vi "measure BT Frequency Separation Step2.vi"(8 "error in (no error)":errorcluster, 11 "SA Measurement in":refnum<class "SA Measurement.lvclass">) -> (0 "error out":errorcluster, 3 "SA Measurement out":refnum<class "SA Measurement.lvclass">)   [LabVIEW 2023, in "Spectrum Analyzer.lvlib" / "SA Measurement.lvclass"]
uses:
  SA Measurement.lvclass
  SA Measurement.lvclass/SA Measurement.ctl
  TYPE DEFINITION/TYPE Marker Peak Search Type.ctl
  Spectrum Analyzer.lvlib
  Interface_Spectrum/Interface_Spectrum.lvclass
  TYPE DEFINITION/TYPE Marker Control Mode.ctl
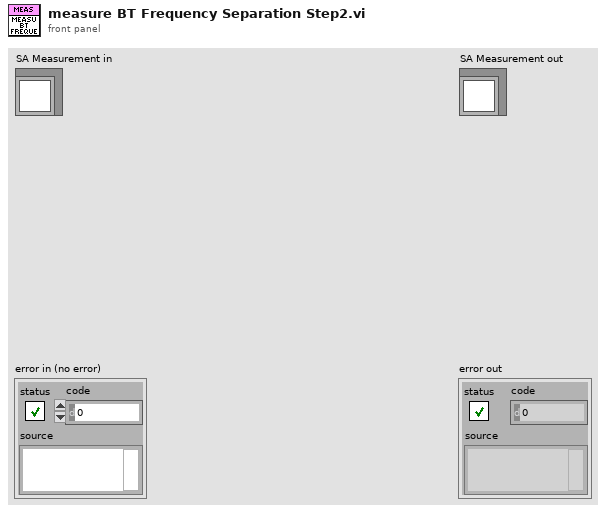
[diagram p1: front panel]
types:
  T1 = typedef "Spectrum Analyzer.lvlib/TYPE Marker Peak Search Type.ctl" = enum16{"Max", "Next Peak"}
  T2 = typedef "Spectrum Analyzer.lvlib/TYPE Marker Control Mode.ctl" = enum16{"Normal", "Delta", "Off"}
  T3 = typedef "Spectrum Analyzer.lvlib/TYPE Marker Value.ctl" = cluster{"X-axis":dbl, "Y-axis":dbl}
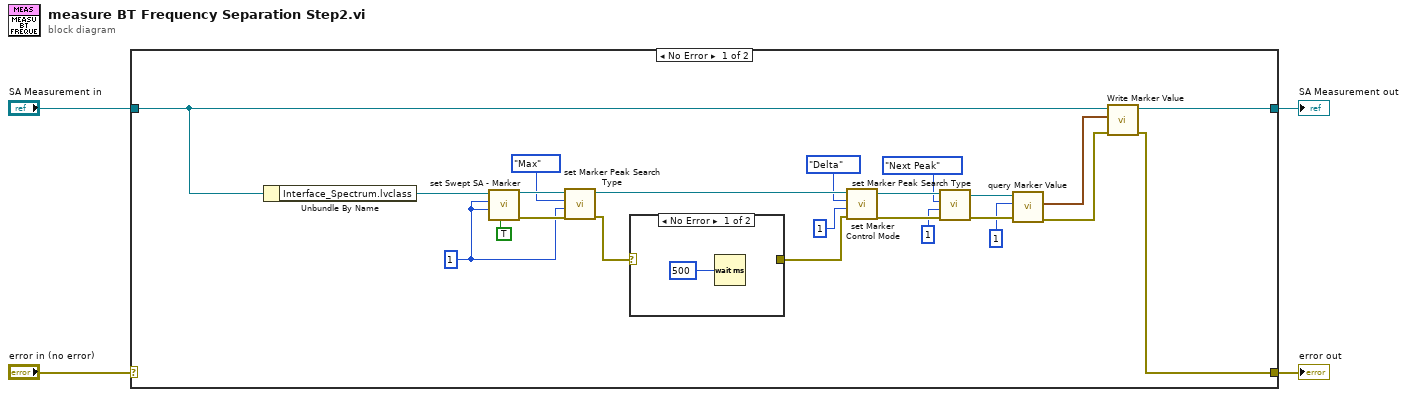
[diagram p0: block diagram]
diagram:
  n1 = case shown="No Error" "error in (no error)" {
    selector: "error in (no error)" -> [_ w31]
    tunnel: [w5 w31] -> w3
    tunnel: [w8 w30] -> w1
    tunnel: "SA Measurement in" -> [w9 w30]
    frame No Error {
      w23 = 1 ("Index")
      n2 = Unbundle By Name(w9) -> ("Interface_Spectrum.lvclass"=w22:refnum<class "Interface_Spectrum.lvclass">)
      n3 = call-dynamic "set Swept SA - Marker.vi"("On?"=TRUE, "trace"=w23, "Index"=w23, "Interface_Spectrum in"=w22) -> ("error out"=w25:errorcluster, "Interface_Spectrum out"=w26:refnum<class "Interface_Spectrum.lvclass">)  [unwired: 6 in]
      n4 = call-dynamic "set Marker Peak Search Type.vi"("error in (no error)"=w25, "Marker Index"=w23, "Peak Search Type"=TYPE_Marker_Peak_Search_Type."Max", "Interface_Spectrum in"=w26) -> ("error out"=w21:errorcluster, "Interface_Spectrum out"=w20:refnum<class "Interface_Spectrum.lvclass">)  [unwired: 6 in]
      n5 = case shown="No Error" w21 {
        selector: w21 -> [_ w29]
        tunnel: [_ w29] -> w19
        frame No Error {
          n6 = Wait (ms)(milliseconds to wait=u32 500) -> ()  [unwired: 1 out]
        }
        frame Error {
        }
      }
      n7 = call-dynamic "set Marker Control Mode.vi"("error in (no error)"=w19, "Marker Index"=1, "Marker Mode"=TYPE_Marker_Control_Mode."Delta", "Interface_Spectrum in"=w20) -> ("error out"=w15:errorcluster, "Interface_Spectrum out"=w16:refnum<class "Interface_Spectrum.lvclass">)  [unwired: 6 in]
      n8 = call-dynamic "set Marker Peak Search Type.vi"("error in (no error)"=w15, "Marker Index"=1, "Peak Search Type"=TYPE_Marker_Peak_Search_Type."Next Peak", "Interface_Spectrum in"=w16) -> ("error out"=w11:errorcluster, "Interface_Spectrum out"=w12:refnum<class "Interface_Spectrum.lvclass">)  [unwired: 6 in]
      n9 = call-dynamic "query Marker Value.vi"("error in (no error)"=w11, "Marker Index"=1, "Interface_Spectrum in"=w12) -> ("error out"=w6:errorcluster, "Marker Value"=w7:T3)  [unwired: 6 in, 1 out]
      n10 = call "Write Marker Value.vi"("error in (no error)"=w6, "Marker Value"=w7, "SA Measurement in"=w9) -> ("error out"=w5:errorcluster, "SA Measurement out"=w8:refnum<class "SA Measurement.lvclass">)  [unwired: 7 in]
    }
    frame Error {
    }
  }
  "error out" <- w3
  "SA Measurement out" <- w1
